vi "A_Loop_Inverted.vi"(4 "N per point":i32, 6 "Tset setting":dbl, 7 "x":dbl, 8 "Numeric 4":dbl, 9 "Numeric 3":i32, 10 "Numeric 2":i32, 11 "Numeric":i32) -> (1 "Array 3":string[](array[string]), 2 "output array 2":string[](array[string]), 3 "output array":string[](array[string]))   [LabVIEW 2024]
panel:
  out "Array 2":string[](array[string])
  out "Array":string[](array[string])
  out "Slide":dbl(slide) scale=0.1..100.0
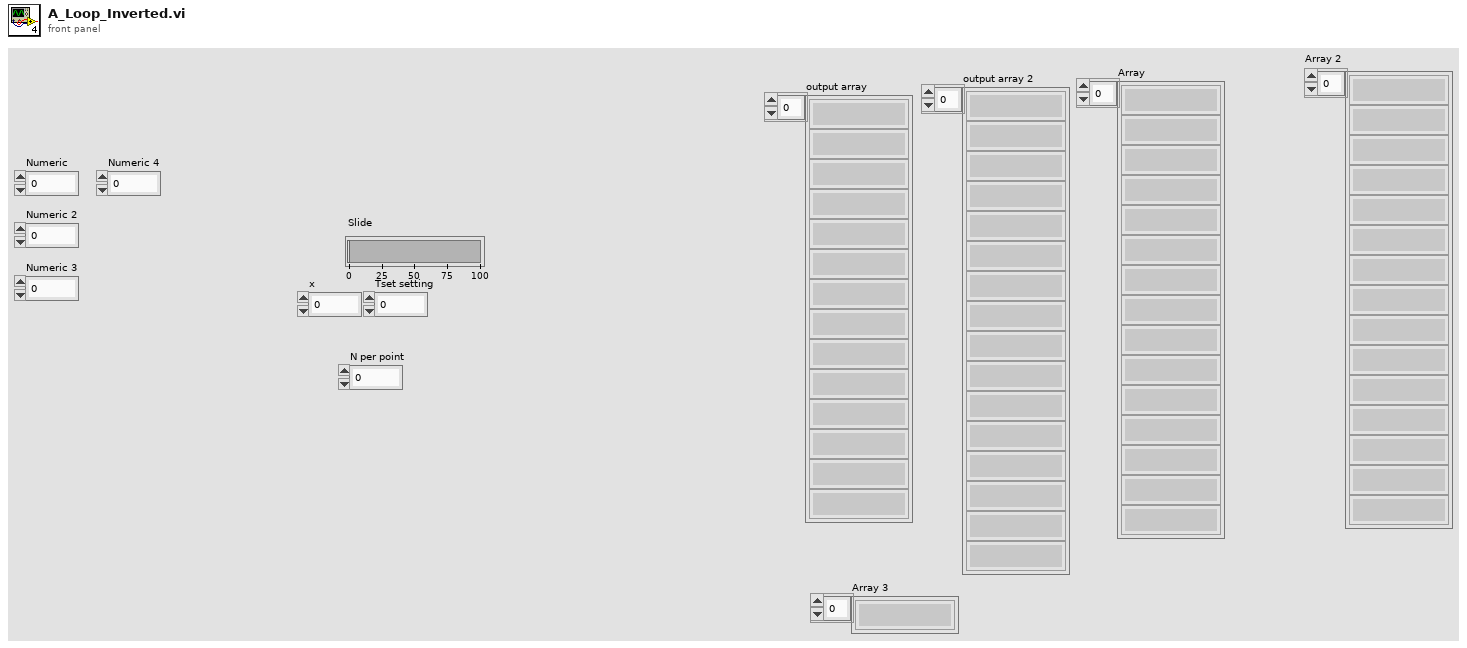
[diagram p1: front panel]
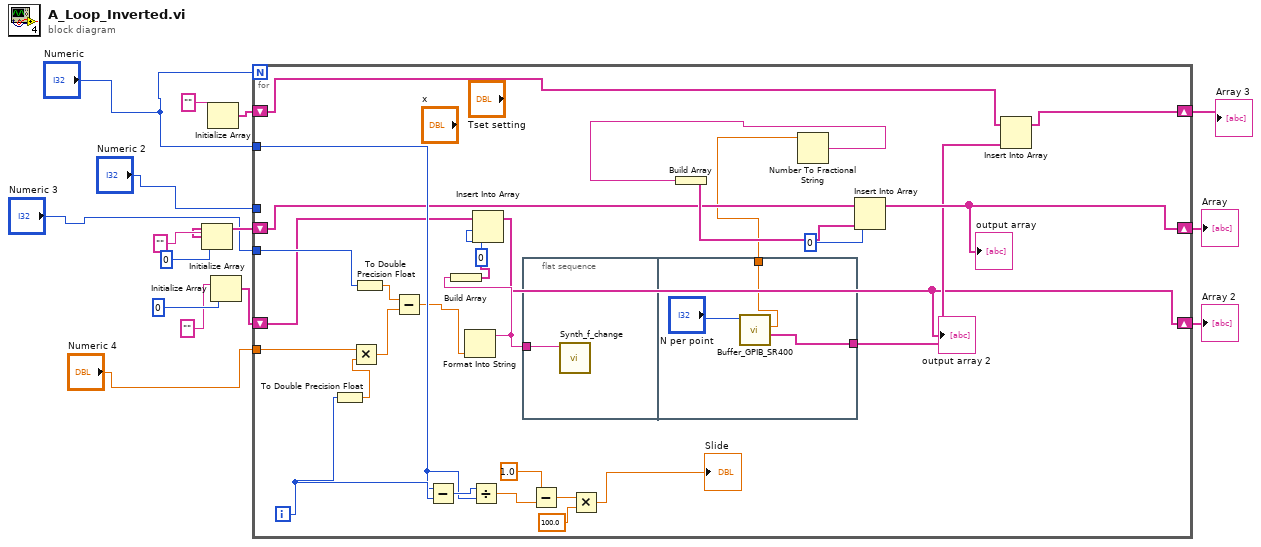
[diagram p0: block diagram]
diagram:
  n1 = Initialize Array("", 0 ("dimension size")) -> (w11:string[])
  n2 = Initialize Array("") -> (w2:string[])  [unwired: 1 in]
  n3 = Initialize Array("", 0 ("dimension size")) -> (w10:string[])
  n4 = for {
    N: "Numeric" -> [_]
    tunnel: "Numeric 4" -> [w43]
    tunnel: "Numeric 2" -> [_]
    tunnel: "Numeric" -> [w36]
    tunnel: "Numeric 3" -> [w24]
    shift-right: [w26] -> w9
    shift-left: w11 -> [w27]
    shift-right: [w16] -> w8
    shift-left: w10 -> [w19]
    shift-right: [w22] -> w1
    shift-left: w2 -> [w23]
    i -> [w38]
    n5 = To Double Precision Float(number=w38) -> (double precision float=w42:dbl)
    n6 = Multiply(x=w43, y=w42) -> (x*y=w28:dbl)
    n7 = To Double Precision Float(number=w24) -> (double precision float=w29:dbl)
    n8 = Subtract(x=w29, y=w28) -> (x-y=w30:dbl)
    n9 = Subtract(x=w36, y=w38) -> (x-y=w37:i32)
    n10 = Format Into String(w30) -> (resulting string=w39:string)  [unwired: 3 in, 1 out]
    n11 = Build Array(w39) -> (w17:string[])
    n12 = Divide(x=w37, y=w36) -> (x/y=w34:dbl)
    n13 = Insert Into Array "Insert Into Array"(array=w19, index=0 ("index (row)"), new element=w17) -> (w16:string[])
    "output array 2" <- w16
    n14 = flat-sequence {
      tunnel: w39 -> [w44]
      tunnel: [w47] -> w21
      tunnel: [w46] -> w20
      frame #0 {
        n15 = call "Synth_f_change.vi"("string"=w44) -> ()  [unwired: 11 in]
      }
      frame #1 {
        n16 = call "Buffer_GPIB_SR400.vi"("N per point"="N per point") -> ("Array"=w47:string[], "x/y"=w46:dbl)  [unwired: 9 in]
      }
    }
    n17 = Subtract(x=1.0, y=w34) -> (x-y=w33:dbl)
    n18 = Multiply(x=w33, y=100.0) -> (x*y=→"Slide":dbl)
    n19 = Number To Fractional String(number=w20) -> (F-format string=w31:string)  [unwired: 3 in]
    n20 = Build Array(w31) -> (w41:string[])
    n21 = Insert Into Array "Insert Into Array"(array=w27, index=0, new element=w41) -> (w26:string[])
    "output array" <- w26
    n22 = Insert Into Array(array=w23, new element=w21) -> (w22:string[])  [unwired: 1 in]
  }
  "Array" <- w9
  "Array 2" <- w8
  "Array 3" <- w1
